vi "DUT Bringup Search for correct digipat File.vi"(8 "DUT Bring Up Pattern name":string, 10 "DPE Project Path":path) -> (3 "DUT Bring Up .digipat File":path)   [LabVIEW 2025, in "Digital Pattern Sequencer.lvclass"]
uses:
  Digital Pattern Sequencer.lvclass
  Digital Pattern Sequencer.lvclass/Digital Pattern Sequencer.ctl
panel:
  out "Correct .digipat?":bool
  out "error out":errorcluster
  out "Pattern Name":string
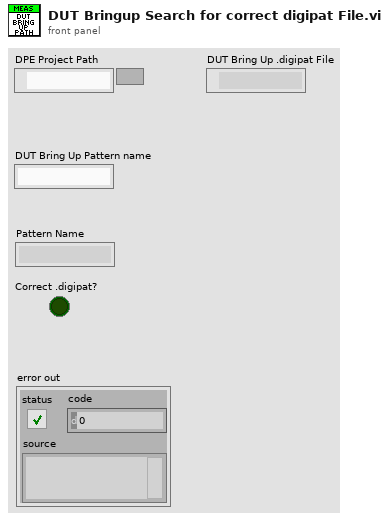
[diagram p1: front panel]
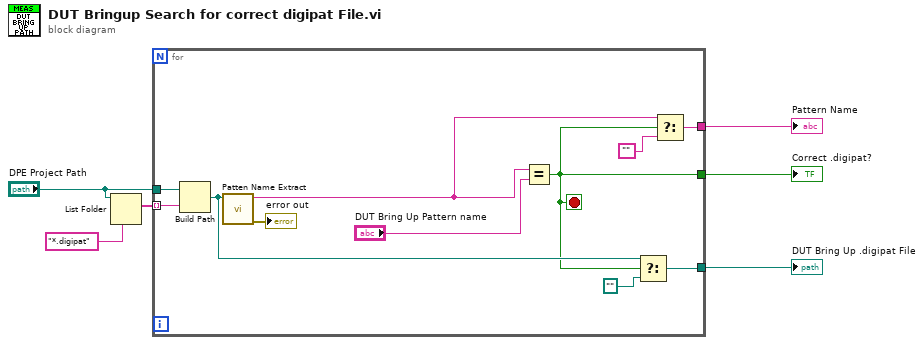
[diagram p0: block diagram]
diagram:
  n1 = List Folder(path="DPE Project Path", pattern="*.digipat") -> (filenames=w4:string[])  [unwired: 2 in, 3 out]
  n2 = for {
    tunnel: [w9] -> w6
    tunnel: w4 -> [w15] mode=indexing
    tunnel: "DPE Project Path" -> [w14]
    tunnel: [w11] -> w2
    tunnel: [w8] -> w1
    stop <- w8 stop-if-true
    n3 = Build Path(base path=w14, name or relative path=w15) -> (appended path=w13:path)
    n4 = call "Patten Name Extract.vi"("Digipat source file"=w13) -> ("error out"=→"error out":errorcluster, "pattern name"=w12:string)  [unwired: 9 in]
    n5 = Equal?(x=w12, y="DUT Bring Up Pattern name") -> (x = y?=w8:bool)
    n6 = Select(t=w13, s=w8, f=path "") -> (s? t:f=w9:path)
    n7 = Select(t=w12, s=w8, f="") -> (s? t:f=w11:string)
  }
  "DUT Bring Up .digipat File" <- w6
  "Pattern Name" <- w2
  "Correct .digipat?" <- w1
